vi "Module Init.vi"(8 "error in (no error)":errorcluster, 11 "ValveControlModule in":refnum<class "DigitalControlModule.lvclass">) -> (0 "error out":errorcluster, 3 "ValveControlModule out":refnum<class "DigitalControlModule.lvclass">)   [LabVIEW 2020, in "VolatusControl.lvlib" / "DigitalControlModule.lvclass"]
uses:
  DigitalControlModule.lvclass
  DigitalControlModule.lvclass/DigitalControlModule.ctl
  lv-cdm/CDM-Config/Config Element/Config Element.lvclass
  Volatus/Module/Module.lvclass
  Volatus/Message Registration.ctl
  Volatus/Volatus.lvlib
  VolatusConfig/Group/Group Config.lvclass
  lv-vecto/Vecto/Group DBL/Group DBL.lvclass
  VolatusData/Data Processor Module/Data Processor Module.lvclass
  C:/dev/lv20CE/relink/lv-volatus/Volatus/Module/Module.lvclass
  C:/dev/lv20CE/relink/lv-volatus/VolatusControl/DigitalControlModule/DigitalControlModule.lvclass
  VolatusConfig/VolatusConfigElement/VolatusConfigElement.lvclass
  VolatusConfig/VolatusConfig.lvlib
  VolatusConfig/Meta Type.ctl
  VolatusData/Data Buffer DBL/Data Buffer DBL.lvclass
  C:/dev/lv20CE/relink/lv-vecto/Vecto/Group/Group.lvclass
  C:/dev/lv20CE/relink/lv-vecto/Vecto/Group DBL/Group DBL.lvclass
  lv-vecto/Vecto/Group/Group.lvclass
  VolatusConfig/Task/Task Config.lvclass
  C:/dev/lv20CE/relink/lv-volatus/VolatusConfig/VolatusConfigElement/VolatusConfigElement.lvclass
  C:/dev/lv20CE/relink/lv-volatus/VolatusConfig/Task/Task Config.lvclass
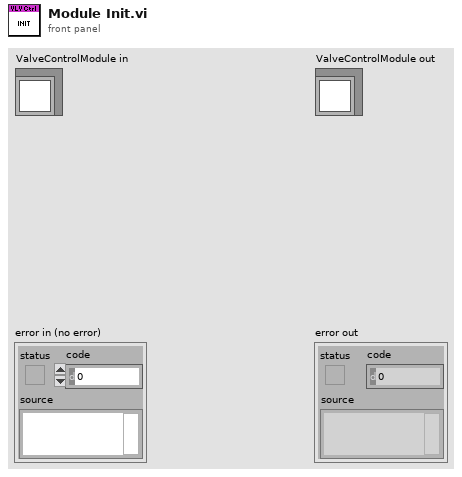
[diagram p1: front panel]
types:
  T1 = typedef "VolatusConfig.lvlib/Meta Type.ctl" = enum16{"UNKNOWN", "VL_System", "VL_Cluster", "VL_Node", "VL_Task", "VL_Group", "VL_Channel", "VL_Task_List", "VL_Scaling", "VL_Sensor", "VL_Sensor_List", "VL_Scale"}
  T2 = typedef "Volatus.lvlib/Message Registration.ctl" = cluster{"Message Type":string, "Message ID":string}
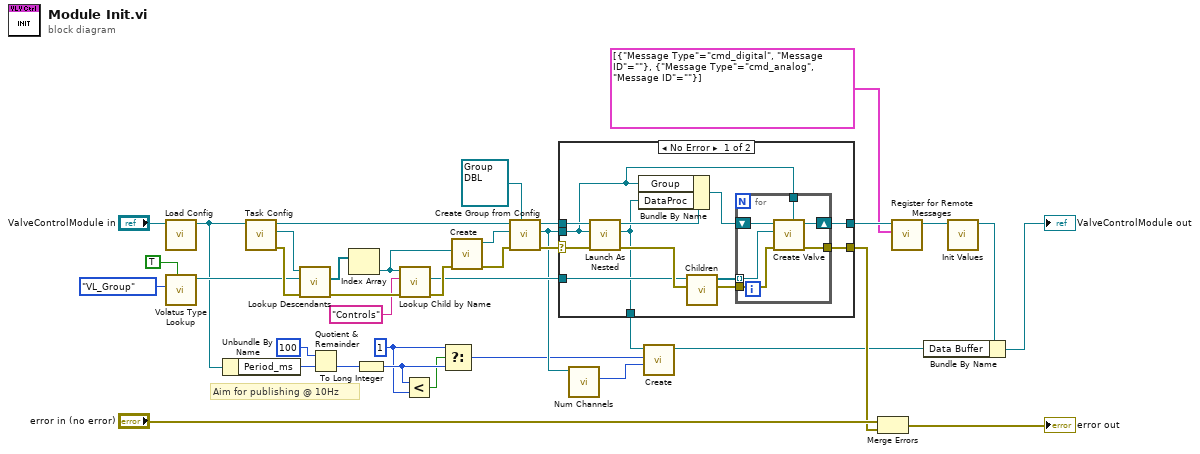
[diagram p0: block diagram]
diagram:
  w3 = 1
  # "Aim for publishing @ 10Hz"
  n1 = call "Load Config.vi"("ValveControlModule in"="ValveControlModule in") -> ("ValveControlModule out"=w14:refnum<class "DigitalControlModule.lvclass">)  [unwired: 9 in, 1 out]
  n2 = call "Volatus Type Lookup.vi"("Don't Recurse Past Match (F)"=TRUE, "Meta Type"=Meta_Type."VL_Group") -> ("Config Lookup out"=w20:refnum<class "Config Lookup.lvclass">)  [unwired: 8 in, 1 out]
  n3 = Unbundle By Name(w14) -> ("Period_ms"=w12:i64)
  n4 = call "Task Config.vi"("Module in"=w14) -> ("error out"=w38:errorcluster, "Task Config"=w30:refnum<class "Task Config.lvclass">, "Module out"=w28:refnum<class "DigitalControlModule.lvclass">)  [unwired: 8 in]
  n5 = call "Lookup Descendants.vi"("error in (no error)"=w38, "Lookup"=w20, "VolatusConfigElement in"=w30) -> ("error out"=w36:errorcluster, "Descendants"=w29:refnum<class "Config Element.lvclass">[])  [unwired: 6 in, 1 out]
  n6 = Quotient & Remainder(x=i64 100, y=w12) -> (floor(x/y)=w11:i64)  [unwired: 1 out]
  n7 = Index Array(array=w29) -> (element=w17:refnum<class "Config Element.lvclass">)  [unwired: 1 in]
  n8 = To Long Integer(number=w11) -> (32bit integer=w4:i32)
  n9 = call "Lookup Child by Name.vi"("error in (no error)"=w36, "Name"="Controls", "Config Element in"=w17) -> ("error out"=w37:errorcluster, "Child"=w15:refnum<class "Config Element.lvclass">)  [unwired: 5 in, 2 out]
  n10 = Less?(x=w4, y=w3) -> (x < y?=w2:bool)
  n11 = Select(t=w3, s=w2, f=w4) -> (s? t:f=w1:i32)
  n12 = call "Create.vi"("error in (no error)"=w37, "Element"=w17) -> ("error out"=w26:errorcluster, "Group out"=w27:refnum<class "Group Config.lvclass">)  [unwired: 8 in]
  n13 = call "Create Group from Config.vi"("Group Type (Abstract)"=refnum<class "Group DBL.lvclass"> refnum ("Vecto.lvlib:Group.lvclass"), "error in (no error)"=w26, "Group Config"=w27, "Module in"=w28) -> ("error out"=w22:errorcluster, "Group"=w9:refnum<class "Group DBL.lvclass">, "Module out"=w23:refnum<class "DigitalControlModule.lvclass">)  [unwired: 5 in]
  n14 = case shown="No Error" w22 {
    selector: w22 -> [w41 w57]
    tunnel: [w47 w57] -> w32
    tunnel: w15 -> [w46 _]
    tunnel: [w45 w58] -> w24
    tunnel: w9 -> [w40 _]
    tunnel: w23 -> [w44 w58]
    tunnel: [w39 _] -> w10
    frame No Error {
      n15 = call "Launch As Nested.vi"("error in (no error)"=w41, "Group"=w40, "Parent in"=w44) -> ("error out"=w50:errorcluster, "MessageQ"=w39:refnum<class "MessageQ.lvclass">, "Parent out"=w43:refnum<class "DigitalControlModule.lvclass">)  [unwired: 6 in]
      n16 = Bundle By Name(cluster=w43, "Group"=w40, "DataProc"=w39) -> (w42:refnum<class "DigitalControlModule.lvclass">)
      n17 = call "Children.vi"("error in (no error)"=w50, "Config Element in"=w46) -> ("error out"=w48:errorcluster, "Elements"=w49:refnum<class "Config Element.lvclass">[])  [unwired: 8 in]
      n18 = for {
        tunnel: w49 -> [w55] mode=indexing
        shift-right: [w54] -> w45
        shift-left: w42 -> [w56]
        tunnel: w48 -> [w53]
        tunnel: [w52] -> w47
        tunnel: w40 -> [w51]
        n19 = call "Create Valve.vi"("Group"=w51, "error in (no error)"=w53, "Config Element"=w55, "ValveControlModule in"=w56) -> ("error out"=w52:errorcluster, "ValveControlModule out"=w54:refnum<class "DigitalControlModule.lvclass">)  [unwired: 6 in]
      }
    }
    frame Error {
    }
  }
  n20 = call "Num Channels.vi"("GroupAbstract in"=w9) -> ("Num Channels"=w8:i32)  [unwired: 8 in, 2 out]
  n21 = call "Create.vi"("# Chans"=w8, "Size"=w1, "MsgQ"=w10) -> ("Data Buffer out"=w7:refnum<class "Data Buffer DBL.lvclass">)  [unwired: 7 in, 1 out]
  n22 = Merge Errors("error in (no error)", w32) -> (→"error out":errorcluster)
  n23 = call "Register for Remote Messages.vi"("Messages"=T2[] [{"Message Type"="cmd_digital", "Message ID"=""}, {"Message Type"="cmd_analog", "Message ID"=""}], "Module in"=w24) -> ("Module out"=w31:refnum<class "DigitalControlModule.lvclass">)  [unwired: 8 in, 1 out]
  n24 = call "Init Values.vi"("ValveControlModule in"=w31) -> ("ValveControlModule out"=w6:refnum<class "DigitalControlModule.lvclass">)  [unwired: 9 in, 1 out]
  n25 = Bundle By Name(cluster=w6, "Data Buffer"=w7) -> (→"ValveControlModule out":refnum<class "DigitalControlModule.lvclass">)
